vi "Read Pin Map File Contents.vi"(8 "error in":errorcluster, 11 "pin map file path":path) -> (0 "error out":errorcluster, 3 "pin map xml":string)   [LabVIEW 2021, in "NI Pin Map V1 Client.lvlib"]
uses:
  NI Pin Map V1 Client.lvlib
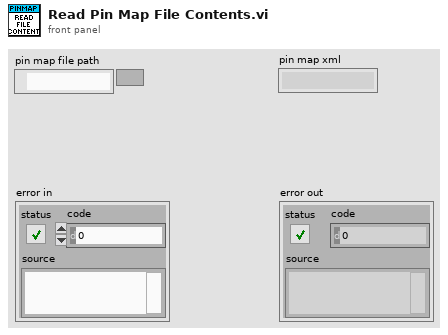
[diagram p1: front panel]
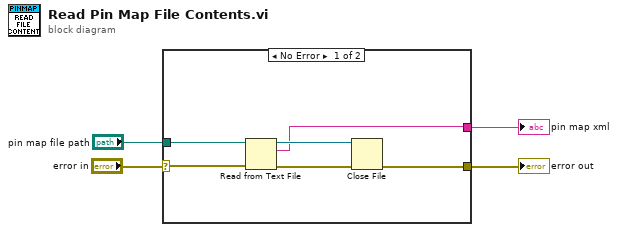
[diagram p0: block diagram]
diagram:
  n1 = case shown="No Error" "error in" {
    selector: "error in" -> [w10 w11]
    tunnel: "pin map file path" -> [w9 _]
    tunnel: [w6 w11] -> w1
    tunnel: [w5 _] -> w2
    frame No Error {
      n2 = Read from Text File(file (use dialog)=w9, error in=w10) -> (refnum out=w8:refnum<file>, text=w5:string, error out=w7:errorcluster)  [unwired: 2 in, 1 out]
      n3 = Close File(refnum=w8, error in=w7) -> (error out=w6:errorcluster)  [unwired: 1 out]
    }
    frame Error {
    }
  }
  "pin map xml" <- w2
  "error out" <- w1
